vi "measure BT Power.vi"(8 "error in (no error)":errorcluster, 11 "SA Measurement in":refnum<class "SA Measurement.lvclass">) -> (0 "error out":errorcluster, 2 "Channel Power":dbl, 3 "SA Measurement out":refnum<class "SA Measurement.lvclass">)   [LabVIEW 2023, in "Spectrum Analyzer.lvlib" / "SA Measurement.lvclass"]
uses:
  SA Measurement.lvclass
  SA Measurement.lvclass/SA Measurement.ctl
  TYPE DEFINITION/Keysight 9020A/TYPE Measurement Preset.ctl
  Spectrum Analyzer.lvlib
  TYPE DEFINITION/TYPE RBW and VBW Select.ctl
  Interface_Spectrum/Interface_Spectrum.lvclass
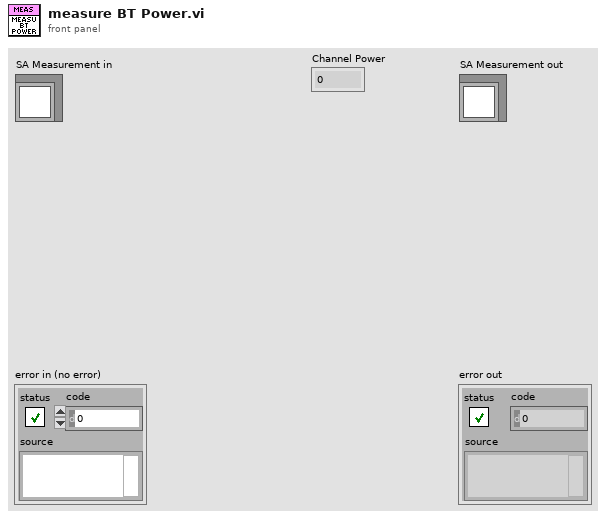
[diagram p1: front panel]
types:
  T1 = typedef "Spectrum Analyzer.lvlib/TYPE RBW and VBW Select.ctl" = enum16{"Res BW", "Video BW"}
  T2 = typedef "Spectrum Analyzer.lvlib/TYPE Measurement Preset.ctl" = enum16{"Sweep SA Mode", "Channel Power", "Occupied BW", "ACP", "Spurious Emission", "Spurious Emission Mask", "Burst Power (Transmit Power)"}
  T3 = typedef "Spectrum Analyzer.lvlib/TYPE Reference Level and Atten Param.ctl" = cluster{"Reference Level":dbl, "Atten":i32, "Atten Auto?":bool, "Reference Level Offset":dbl}
  T4 = typedef "Spectrum Analyzer.lvlib/TYPE Display Trace Mode Select.ctl" = enum16{"Clear Write", "Max Hold", "Min Hold", "Average", "View"}
  T5 = typedef "Spectrum Analyzer.lvlib/TYPE Detect Mode Select.ctl" = enum16{"Det Auto (Normal)", "Auto Peak", "Positive Peak", "Negative Peak", "Sample", "RMS", "Average", "Quasipeak", "CISPR Average", "RMS Average"}
  T6 = cluster{"Trace Mode":T4, "Detector Type":T5, "Detect Auto?":bool}[]
  T7 = enum16{"External 1", "External 2", "Line", "Frame", "RF Burst", "TV", "PXI"}
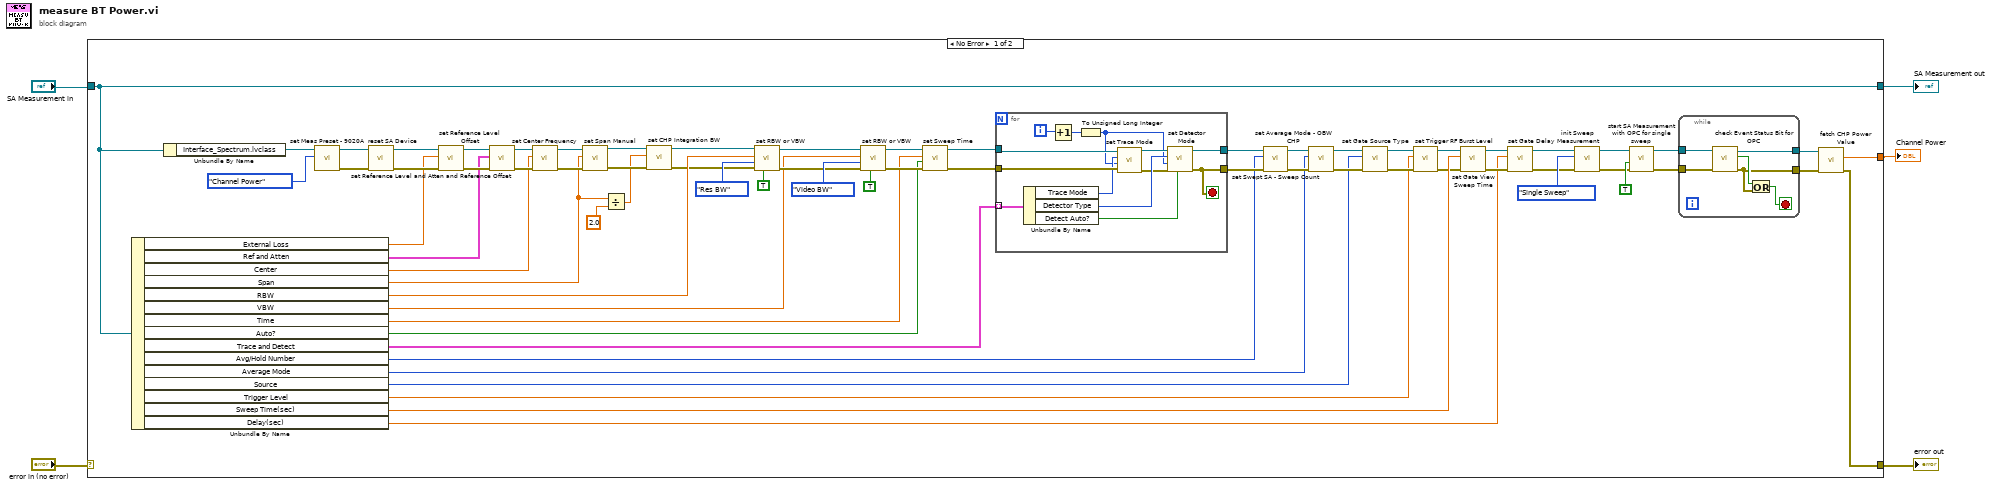
[diagram p0: block diagram]
diagram:
  n1 = case shown="No Error" "error in (no error)" {
    selector: "error in (no error)" -> [_ w94]
    tunnel: [w7 w94] -> w2
    tunnel: [w50 w93] -> w3
    tunnel: "SA Measurement in" -> [w50 w93]
    tunnel: [w6 _] -> w1
    frame No Error {
      n2 = Unbundle By Name(w50) -> ("External Loss"=w65:dbl, "Ref and Atten"=w64:T3, "Center"=w47:dbl, "Span"=w33:dbl, "RBW"=w57:dbl, "VBW"=w56:dbl, "Time"=w42:dbl, "Auto?"=w41:bool, "Trace and Detect"=w55:T6, "Avg/Hold Number"=w52:u32, "Average Mode"=w36:enum16{"Exponential", "Repeat"}, "Source"=w26:T7, "Trigger Level"=w19:dbl, "Sweep Time(sec)"=w25:dbl, "Delay(sec)"=w22:dbl)
      n3 = Unbundle By Name(w50) -> ("Interface_Spectrum.lvclass"=w73:refnum<class "Interface_Spectrum.lvclass">)
      n4 = call-dynamic "set Meas Preset - 9020A.vi"("Measurement Preset"=TYPE_Measurement_Preset."Channel Power", "Interface_Spectrum in"=w73) -> ("error out"=w70:errorcluster, "Interface_Spectrum out"=w71:refnum<class "Interface_Spectrum.lvclass">)  [unwired: 8 in]
      n5 = call-dynamic "reset SA Device.vi"("error in (no error)"=w70, "Interface_Spectrum in"=w71) -> ("error out"=w68:errorcluster, "Interface_Spectrum out"=w69:refnum<class "Interface_Spectrum.lvclass">)  [unwired: 8 in]
      n6 = call-dynamic "set Reference Level Offset.vi"("error in (no error)"=w68, "Reference Level Offset"=w65, "Interface_Spectrum in"=w69) -> ("error out"=w66:errorcluster, "Interface_Spectrum out"=w67:refnum<class "Interface_Spectrum.lvclass">)  [unwired: 7 in]
      n7 = call-dynamic "set Reference Level and Atten and Reference Offset.vi"("error in (no error)"=w66, "Reference Level, Atten, Reference Offset"=w64, "Interface_Spectrum in"=w67) -> ("error out"=w48:errorcluster, "Interface_Spectrum out"=w49:refnum<class "Interface_Spectrum.lvclass">)  [unwired: 7 in]
      n8 = call-dynamic "set Center Frequency.vi"("error in (no error)"=w48, "Center Frequency (Hz)"=w47, "Interface_Spectrum in"=w49) -> ("error out"=w45:errorcluster, "Interface_Spectrum out"=w46:refnum<class "Interface_Spectrum.lvclass">)  [unwired: 7 in]
      n9 = call-dynamic "set Span Manual.vi"("error in (no error)"=w45, "Span (Hz)"=w33, "Interface_Spectrum in"=w46) -> ("error out"=w34:errorcluster, "Interface_Spectrum out"=w35:refnum<class "Interface_Spectrum.lvclass">)  [unwired: 7 in]
      n10 = Divide(x=w33, y=2.0) -> (x/y=w31:dbl)
      n11 = call-dynamic "set CHP Integration BW.vi"("error in (no error)"=w34, "Integration BW (Hz)"=w31, "Interface_Spectrum in"=w35) -> ("error out"=w29:errorcluster, "Interface_Spectrum out"=w30:refnum<class "Interface_Spectrum.lvclass">)  [unwired: 7 in]
      n12 = call-dynamic "set RBW or VBW.vi"("BW Auto?"=TRUE, "error in (no error)"=w29, "BW Type"=TYPE_RBW_and_VBW_Select."Res BW", "BW Value (Hz)"=w57, "Interface_Spectrum in"=w30) -> ("error out"=w58:errorcluster, "Interface_Spectrum out"=w59:refnum<class "Interface_Spectrum.lvclass">)  [unwired: 5 in]
      n13 = call-dynamic "set RBW or VBW.vi"("BW Auto?"=TRUE, "error in (no error)"=w58, "BW Type"=TYPE_RBW_and_VBW_Select."Video BW", "BW Value (Hz)"=w56, "Interface_Spectrum in"=w59) -> ("error out"=w43:errorcluster, "Interface_Spectrum out"=w44:refnum<class "Interface_Spectrum.lvclass">)  [unwired: 5 in]
      n14 = call-dynamic "set Sweep Time.vi"("error in (no error)"=w43, "Sweep Time Auto?"=w41, "Sweep Time(sec)"=w42, "Interface_Spectrum in"=w44) -> ("error out"=w39:errorcluster, "Interface_Spectrum out"=w40:refnum<class "Interface_Spectrum.lvclass">)  [unwired: 6 in]
      n15 = for {
        tunnel: w40 -> [w91]
        tunnel: w39 -> [w90]
        tunnel: w55 -> [w92] mode=indexing
        tunnel: [w80] -> w53
        tunnel: [w81] -> w54
        i -> [w89]
        stop <- w80 stop-if-true
        n16 = Unbundle By Name(w92) -> ("Trace Mode"=w87:T4, "Detector Type"=w85:T5, "Detect Auto?"=w82:bool)
        n17 = Increment(x=w89) -> (x+1=w88:i32)
        n18 = To Unsigned Long Integer(number=w88) -> (unsigned 32bit integer=w83:u32)
        n19 = call-dynamic "set Trace Mode.vi"("error in (no error)"=w90, "Trace Index"=w83, "Trace Mode"=w87, "Interface_Spectrum in"=w91) -> ("error out"=w84:errorcluster, "Interface_Spectrum out"=w86:refnum<class "Interface_Spectrum.lvclass">)  [unwired: 6 in]
        n20 = call-dynamic "set Detector Mode.vi"("Detect Auto?"=w82, "error in (no error)"=w84, "Trace Index"=w83, "Detector Type"=w85, "Interface_Spectrum in"=w86) -> ("error out"=w80:errorcluster, "Interface_Spectrum out"=w81:refnum<class "Interface_Spectrum.lvclass">)  [unwired: 5 in]
      }
      n21 = call-dynamic "set Swept SA - Sweep Count.vi"("error in (no error)"=w53, "Sweep Count"=w52, "Interface_Spectrum in"=w54) -> ("error out"=w37:errorcluster, "Interface_Spectrum out"=w38:refnum<class "Interface_Spectrum.lvclass">)  [unwired: 7 in]
      n22 = call-dynamic "set Average Mode - OBW CHP.vi"("error in (no error)"=w37, "Average Mode"=w36, "Interface_Spectrum in"=w38) -> ("error out"=w27:errorcluster, "Interface_Spectrum out"=w28:refnum<class "Interface_Spectrum.lvclass">)  [unwired: 7 in]
      n23 = call-dynamic "set Gate Source Type.vi"("error in (no error)"=w27, "Gate Source"=w26, "Interface_Spectrum in"=w28) -> ("error out"=w20:errorcluster, "Interface_Spectrum out"=w21:refnum<class "Interface_Spectrum.lvclass">)  [unwired: 7 in]
      n24 = call-dynamic "set Trigger RF Burst Level.vi"("error in (no error)"=w20, "ABS level (dBm)"=w19, "Interface_Spectrum in"=w21) -> ("error out"=w17:errorcluster, "Interface_Spectrum out"=w18:refnum<class "Interface_Spectrum.lvclass">)  [unwired: 7 in]
      n25 = call-dynamic "set Gate View Sweep Time.vi"("error in (no error)"=w17, "View Sweep Time (sec)"=w25, "Interface_Spectrum in"=w18) -> ("error out"=w23:errorcluster, "Interface_Spectrum out"=w24:refnum<class "Interface_Spectrum.lvclass">)  [unwired: 7 in]
      n26 = call-dynamic "set Gate Delay.vi"("error in (no error)"=w23, "Gate Delay Time (sec)"=w22, "Interface_Spectrum in"=w24) -> ("error out"=w15:errorcluster, "Interface_Spectrum out"=w16:refnum<class "Interface_Spectrum.lvclass">)  [unwired: 7 in]
      n27 = call-dynamic "init Sweep Measurement.vi"("error in (no error)"=w15, "Sweep Measurement Mode"=enum16{"Single Sweep", "Continuous Sweep"}."Single Sweep", "Interface_Spectrum in"=w16) -> ("error out"=w12:errorcluster, "Interface_Spectrum out"=w13:refnum<class "Interface_Spectrum.lvclass">)  [unwired: 7 in]
      n28 = call-dynamic "start SA Measurement with OPC for single sweep.vi"("error in (no error)"=w12, "with OPC?"=TRUE, "Interface_Spectrum in"=w13) -> ("error out"=w10:errorcluster, "Interface_Spectrum out"=w11:refnum<class "Interface_Spectrum.lvclass">)  [unwired: 7 in]
      n29 = while {
        tunnel: w11 -> [w79]
        tunnel: w10 -> [w78]
        tunnel: [w75] -> w8
        tunnel: [w74] -> w9
        stop <- w76 stop-if-true
        n30 = call-dynamic "check Event Status Bit for OPC.vi"("error in (no error)"=w78, "Interface_Spectrum in"=w79) -> ("error out"=w75:errorcluster, "OPC Bit Changed?"=w77:bool, "Interface_Spectrum out"=w74:refnum<class "Interface_Spectrum.lvclass">)  [unwired: 7 in]
        n31 = Or(x=w77, y=w75) -> (x .or. y?=w76:bool)
      }
      n32 = call-dynamic "fetch CHP Power Value.vi"("error in (no error)"=w8, "Interface_Spectrum in"=w9) -> ("error out"=w7:errorcluster, "Channel Power"=w6:dbl)  [unwired: 7 in, 1 out]
    }
    frame Error {
    }
  }
  "error out" <- w2
  "SA Measurement out" <- w3
  "Channel Power" <- w1
